vi "VIH Project Tree - Item Tag - Build.vi"(5 "Not found":bool, 7 "cmd (build)":enum16{"build", "init"}(ring), 10 "Item File Path":path, 11 "Item Type":T1) -> (2 "Tree Item Symbol":i32, 3 "Tree Item Tag":string)   [LabVIEW 2014]
doc: "::: VI Helpeks :::\nCopyright (c) 2000-2026 Konstantin Shifershteyn. All rights reserved."
uses:
  VIH Project Tree Typedef - Tree Item Type.ctl
panel:
  # "VI Helpeks\nCopyright (c) 2012-2026 Konstantin Shifershteyn"
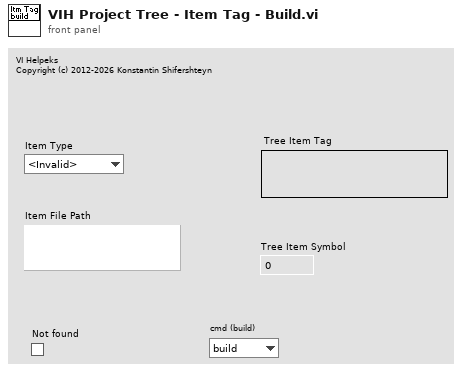
[diagram p1: front panel]
types:
  T1 = typedef "VIH Project Tree Typedef - Tree Item Type.ctl" = enum32{"<Invalid>", "Project", "Proj Files", "Proj Rules", "File Group", "Rule Group", "Any File", "LV Func", ".mnu", ".mnu (dyn)", ".vi", ".vi (dyn)", ".vit", ".vit (dyn)", ".ctl", ".ctl (dyn)", ".ctt", ".ctt (dyn)", "polyVI", "polyVI (dyn)", "expVI", "expVI (dyn)", "HTML", "PolyVI Inst"}
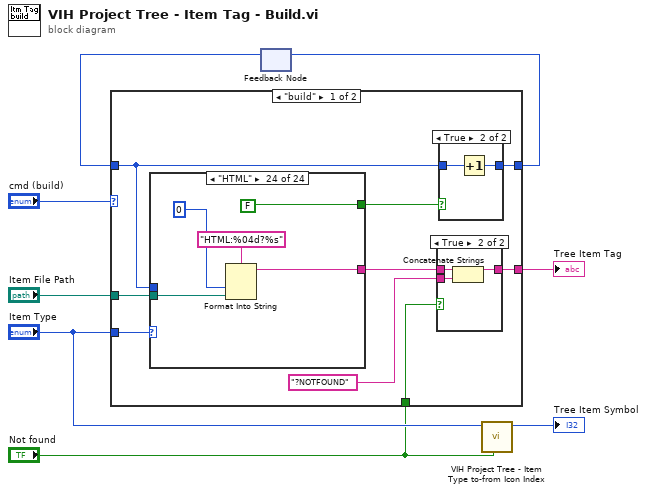
[diagram p0: block diagram]
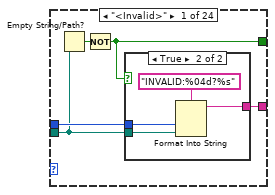
[diagram p4: hidden frame]
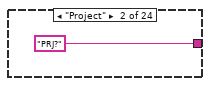
[diagram p6: hidden frame]
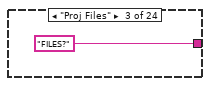
[diagram p7: hidden frame]
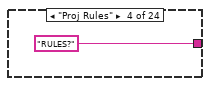
[diagram p8: hidden frame]
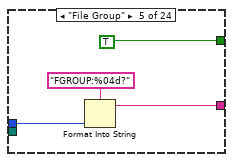
[diagram p9: hidden frame]
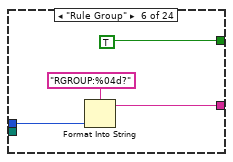
[diagram p10: hidden frame]
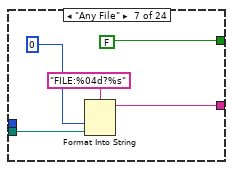
[diagram p11: hidden frame]
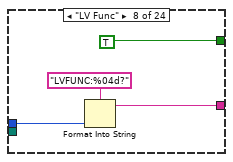
[diagram p12: hidden frame]
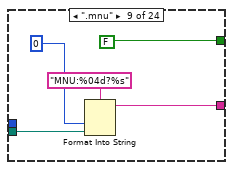
[diagram p13: hidden frame]
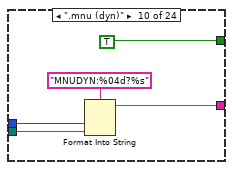
[diagram p14: hidden frame]
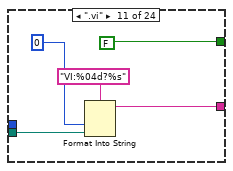
[diagram p15: hidden frame]
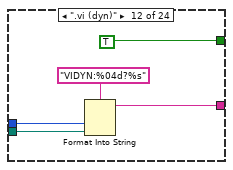
[diagram p16: hidden frame]
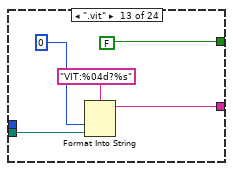
[diagram p17: hidden frame]
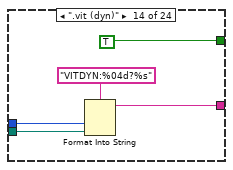
[diagram p18: hidden frame]
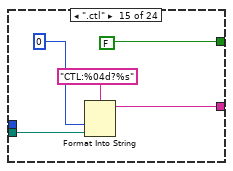
[diagram p19: hidden frame]
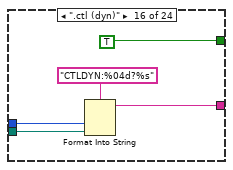
[diagram p20: hidden frame]
diagram:
  n1 = feedback #1() -> (w7:u32)  [unwired: 1 in]
  n2 = case shown="\"build\"" "cmd (build)" {
    tunnel: [w17 u32 1] -> w6
    tunnel: w7 -> [w15 _]
    tunnel: "Item Type" -> [w16 _]
    tunnel: [w11 _] -> w5
    tunnel: "Item File Path" -> [w13 _]
    tunnel: "Not found" -> [w10 _]
    frame "build" {
      n3 = case shown="\"HTML\"" w16 {
        tunnel: [w28 "PRJ?" "FILES?" "RULES?" w40 w44 w49 w53 w58 w63 w68 w73 w78 w83 w88 w93 w98 w103 w108 w113 w118 w123 w128 w133] -> w12
        tunnel: w15 -> [w29 _ _ _ w38 w42 _ w51 _ w61 _ w71 _ w81 _ w91 _ w101 _ w111 w116 _ w126 _]
        tunnel: [w25 _ _ _ TRUE TRUE FALSE TRUE FALSE TRUE FALSE TRUE FALSE TRUE FALSE TRUE FALSE TRUE FALSE TRUE TRUE FALSE TRUE FALSE] -> w14
        tunnel: w13 -> [w27 _ _ _ _ _ w46 _ w55 w59 w65 w69 w75 w79 w85 w89 w95 w99 w105 w109 w114 w120 w124 w130]
        frame "<Invalid>" {
          n4 = Empty String/Path?(string/path=w27) -> (empty?=w26:bool)
          n5 = Not(x=w26) -> (.not. x?=w25:bool)
          n6 = case shown="True" w25 {
            tunnel: w29 -> [_ w32]
            tunnel: [_ w31] -> w28
            tunnel: w27 -> [_ w30]
            frame False {
            }
            frame True {
              n7 = Format Into String(format string="INVALID:%04d?%s", w32, w30) -> (resulting string=w31:string)  [unwired: 2 in, 1 out]
            }
          }
        }
        frame "Project" {
        }
        frame "Proj Files" {
        }
        frame "Proj Rules" {
        }
        frame "File Group" {
          n8 = Format Into String(format string="FGROUP:%04d?", w38) -> (resulting string=w40:string)  [unwired: 2 in, 1 out]
        }
        frame "Rule Group" {
          n9 = Format Into String(format string="RGROUP:%04d?", w42) -> (resulting string=w44:string)  [unwired: 2 in, 1 out]
        }
        frame "Any File" {
          n10 = Format Into String(format string="FILE:%04d?%s", u32 0 ("input 1"), w46) -> (resulting string=w49:string)  [unwired: 2 in, 1 out]
        }
        frame "LV Func" {
          n11 = Format Into String(format string="LVFUNC:%04d?", w51) -> (resulting string=w53:string)  [unwired: 2 in, 1 out]
        }
        frame ".mnu" {
          n12 = Format Into String(format string="MNU:%04d?%s", u32 0 ("input 1"), w55) -> (resulting string=w58:string)  [unwired: 2 in, 1 out]
        }
        frame ".mnu (dyn)" {
          n13 = Format Into String(format string="MNUDYN:%04d?%s", w61, w59) -> (resulting string=w63:string)  [unwired: 2 in, 1 out]
        }
        frame ".vi" {
          n14 = Format Into String(format string="VI:%04d?%s", u32 0 ("input 1"), w65) -> (resulting string=w68:string)  [unwired: 2 in, 1 out]
        }
        frame ".vi (dyn)" {
          n15 = Format Into String(format string="VIDYN:%04d?%s", w71, w69) -> (resulting string=w73:string)  [unwired: 2 in, 1 out]
        }
        frame ".vit" {
          n16 = Format Into String(format string="VIT:%04d?%s", u32 0 ("input 1"), w75) -> (resulting string=w78:string)  [unwired: 2 in, 1 out]
        }
        frame ".vit (dyn)" {
          n17 = Format Into String(format string="VITDYN:%04d?%s", w81, w79) -> (resulting string=w83:string)  [unwired: 2 in, 1 out]
        }
        frame ".ctl" {
          n18 = Format Into String(format string="CTL:%04d?%s", u32 0 ("input 1"), w85) -> (resulting string=w88:string)  [unwired: 2 in, 1 out]
        }
        frame ".ctl (dyn)" {
          n19 = Format Into String(format string="CTLDYN:%04d?%s", w91, w89) -> (resulting string=w93:string)  [unwired: 2 in, 1 out]
        }
        frame ".ctt" {
          n20 = Format Into String(format string="CTT:%04d?%s", u32 0 ("input 1"), w95) -> (resulting string=w98:string)  [unwired: 2 in, 1 out]
        }
        frame ".ctt (dyn)" {
          n21 = Format Into String(format string="CTTDYN:%04d?%s", w101, w99) -> (resulting string=w103:string)  [unwired: 2 in, 1 out]
        }
        frame "polyVI" {
          n22 = Format Into String(format string="POLYVI:%04d?%s", u32 0 ("input 1"), w105) -> (resulting string=w108:string)  [unwired: 2 in, 1 out]
        }
        frame "polyVI (dyn)" {
          n23 = Format Into String(format string="POLYVIDYN:%04d?%s", w111, w109) -> (resulting string=w113:string)  [unwired: 2 in, 1 out]
        }
        frame "PolyVI Inst" {
          n24 = Format Into String(format string="POLYINST:%04d?%s", w116, w114) -> (resulting string=w118:string)  [unwired: 2 in, 1 out]
        }
        frame "expVI" {
          n25 = Format Into String(format string="EXPVI:%04d?%s", u32 0 ("input 1"), w120) -> (resulting string=w123:string)  [unwired: 2 in, 1 out]
        }
        frame "expVI (dyn)" {
          n26 = Format Into String(format string="EXPVIDYN:%04d?%s", w126, w124) -> (resulting string=w128:string)  [unwired: 2 in, 1 out]
        }
        frame "HTML" {
          n27 = Format Into String(format string="HTML:%04d?%s", u32 0 ("input 1"), w130) -> (resulting string=w133:string)  [unwired: 2 in, 1 out]
        }
      }
      n28 = case shown="True" w10 {
        tunnel: w12 -> [w18 w21]
        tunnel: [w18 w20] -> w11
        tunnel: "?NOTFOUND" -> [_ w19]
        frame False {
        }
        frame True {
          n29 = Concatenate Strings(w21, w19) -> (w20:string)
        }
      }
      n30 = case shown="True" w14 {
        tunnel: [w22 w24] -> w17
        tunnel: w15 -> [w22 w23]
        frame False {
        }
        frame True {
          n31 = Increment(x=w23) -> (x+1=w24:u32)
        }
      }
    }
    frame "init" {
    }
  }
  "Tree Item Tag" <- w5
  n32 = feedback-in #1(w6) -> ()
  n33 = call "VIH Project Tree - Item Type to-from Icon Index.vi"("Not found"="Not found", "Item Type"="Item Type") -> ("Icon Index out"=→"Tree Item Symbol":i32)  [unwired: 9 in]
